vi "update CE SEM Mask Table Element.vi"(6 "Mask Type Info":T1, 8 "error in (no error)":errorcluster, 9 "RU Type (0=Full Mask)":i32, 10 "Center Freq":dbl, 11 "SA Measurement in":refnum<class "SA Measurement.lvclass">) -> (0 "error out":errorcluster, 3 "SA Measurement out":refnum<class "SA Measurement.lvclass">)   [LabVIEW 2023, in "Spectrum Analyzer.lvlib" / "SA Measurement.lvclass"]
uses:
  SA Measurement.lvclass
  SA Measurement.lvclass/SA Measurement.ctl
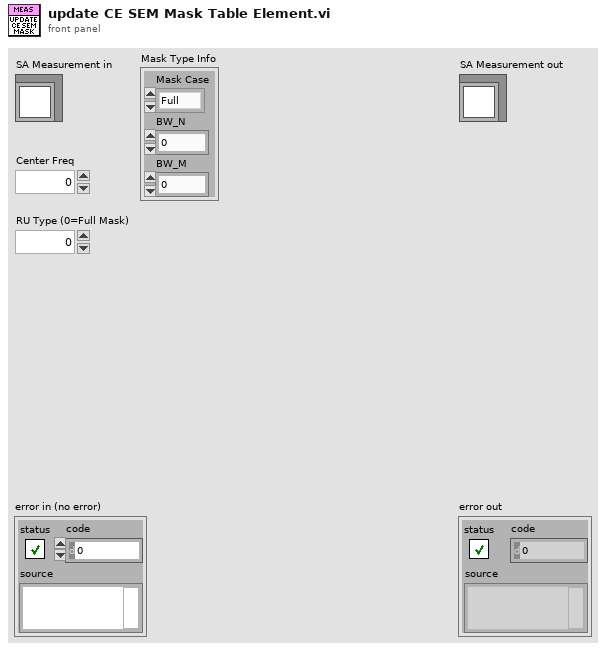
[diagram p1: front panel]
types:
  T1 = cluster{"Mask Case":enum16{"Full", "Case 1", "Case 2", "Case 3", "Case 1+2"}, "BW_N":dbl, "BW_M":dbl}
  T2 = cluster{"Freq":dbl, "Limit":dbl, "dBc Applied?":bool}[]
  T3 = typedef "Spectrum Analyzer.lvlib/TYPE Mask Table for SEM.ctl" = map{enum16{"-10dBm Upper", "-10dBm Lower"}, map{dbl, map{i32, cluster{"Freq":dbl, "Limit":dbl, "dBc Applied?":bool}[]}}}
  T4 = map{dbl, map{i32, cluster{"Freq":dbl, "Limit":dbl, "dBc Applied?":bool}[]}}
  T5 = map{i32, cluster{"Freq":dbl, "Limit":dbl, "dBc Applied?":bool}[]}
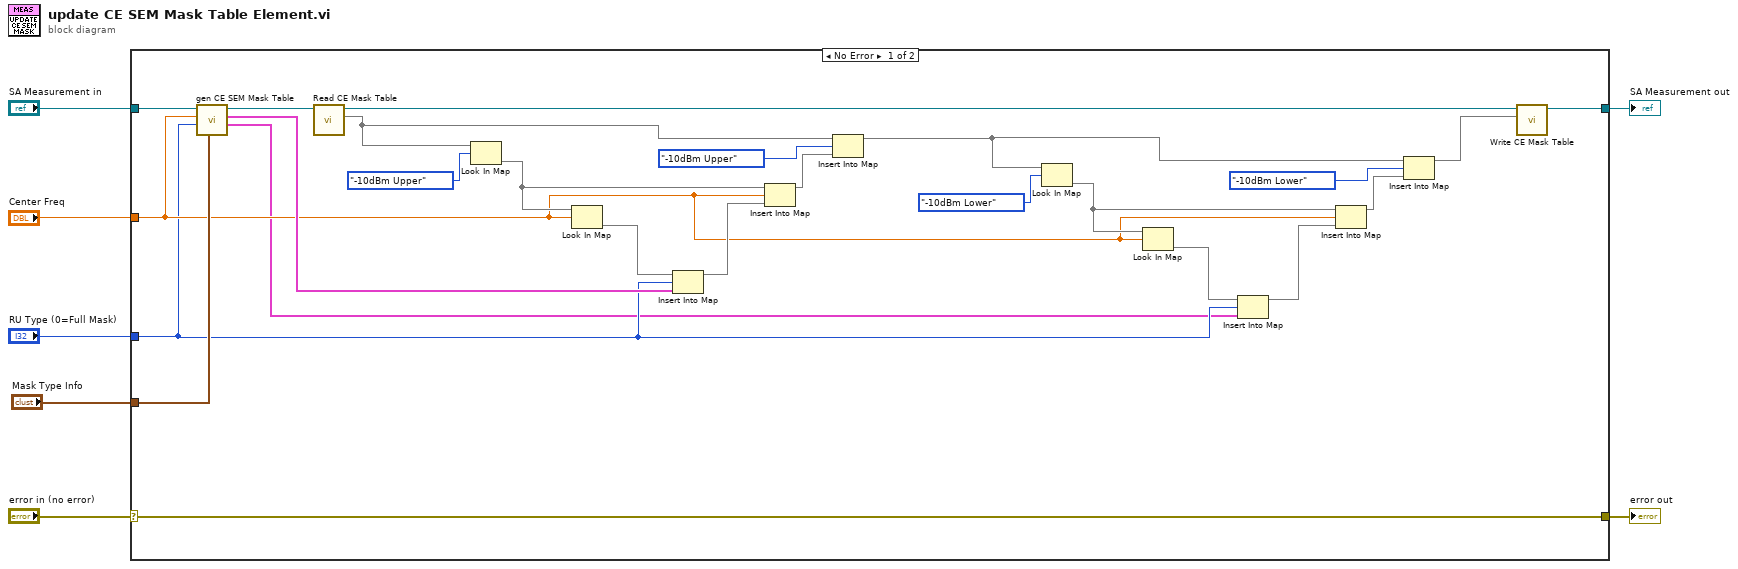
[diagram p0: block diagram]
diagram:
  n1 = case shown="No Error" "error in (no error)" {
    selector: "error in (no error)" -> [w32 w34]
    tunnel: [w32 w34] -> w6
    tunnel: [w28 w33] -> w4
    tunnel: "SA Measurement in" -> [w27 w33]
    tunnel: "Center Freq" -> [w11 _]
    tunnel: "RU Type (0=Full Mask)" -> [w10 _]
    tunnel: "Mask Type Info" -> [w24 _]
    frame No Error {
      n2 = call "gen CE SEM Mask Table.vi"("Mask Type Info"=w24, "RU Type (0=Full Mask)"=w10, "Center Freq"=w11, "SA Measurement in"=w27) -> ("SEM Lower Mask Table"=w9:T2, "SEM Upper Mask Table"=w25:T2, "SA Measurement out"=w26:refnum<class "SA Measurement.lvclass">)  [unwired: 4 in, 1 out]
      n3 = call "Read CE Mask Table.vi"("SA Measurement in"=w26) -> ("Mask Table"=w21:T3, "SA Measurement out"=w29:refnum<class "SA Measurement.lvclass">)  [unwired: 8 in, 1 out]
      n4 = Look In Map(map=w21, key=enum16{"-10dBm Upper", "-10dBm Lower"}."-10dBm Upper") -> (value=w22:T4)  [unwired: 1 in, 1 out]
      n5 = Look In Map(map=w22, key=w11) -> (value=w31:T5)  [unwired: 1 in, 1 out]
      n6 = Insert Into Map(map in=w31, key=w10, value=w25) -> (map out=w30:T5)  [unwired: 2 out]
      n7 = Insert Into Map(map in=w22, key=w11, value=w30) -> (map out=w20:T4)  [unwired: 2 out]
      n8 = Insert Into Map(map in=w21, key=enum16{"-10dBm Upper", "-10dBm Lower"}."-10dBm Upper", value=w20) -> (map out=w12:T3)  [unwired: 2 out]
      n9 = Look In Map(map=w12, key=enum16{"-10dBm Upper", "-10dBm Lower"}."-10dBm Lower") -> (value=w15:T4)  [unwired: 1 in, 1 out]
      n10 = Look In Map(map=w15, key=w11) -> (value=w18:T5)  [unwired: 1 in, 1 out]
      n11 = Insert Into Map(map in=w18, key=w10, value=w9) -> (map out=w17:T5)  [unwired: 2 out]
      n12 = Insert Into Map(map in=w15, key=w11, value=w17) -> (map out=w14:T4)  [unwired: 2 out]
      n13 = Insert Into Map(map in=w12, key=enum16{"-10dBm Upper", "-10dBm Lower"}."-10dBm Lower", value=w14) -> (map out=w8:T3)  [unwired: 2 out]
      n14 = call "Write CE Mask Table.vi"("Mask Table"=w8, "SA Measurement in"=w29) -> ("SA Measurement out"=w28:refnum<class "SA Measurement.lvclass">)  [unwired: 8 in, 1 out]
    }
    frame Error {
    }
  }
  "error out" <- w6
  "SA Measurement out" <- w4
